vi "target_finder_3.vi"(6 "prev_count":i32, 9 "Lane_center":dbl, 10 "roi_dead":bool, 11 "Lane_center in":dbl) -> (1 "next_count":i32, 2 "Reset_ROI":dbl, 3 "Lane_center out":dbl)   [LabVIEW 2024]
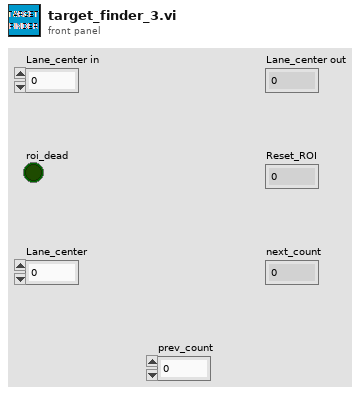
[diagram p1: front panel]
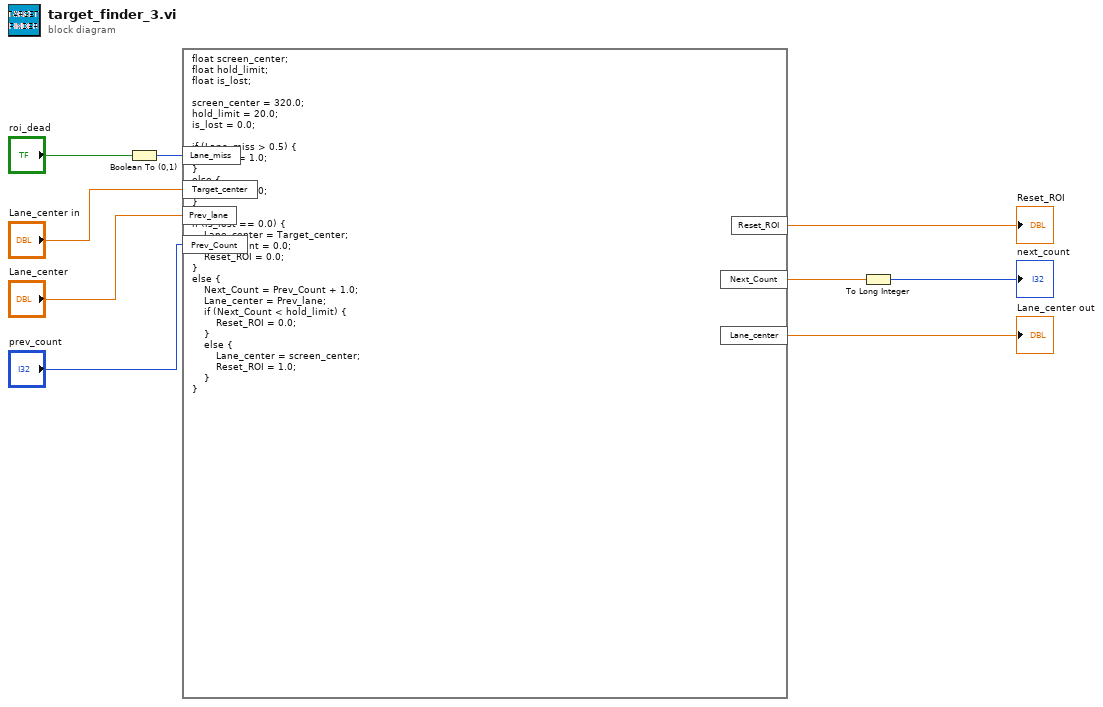
[diagram p0: block diagram]
diagram:
  n1 = Boolean To (0,1)(Boolean="roi_dead") -> (0, 1=w4:i16)
  n2 = formula code="float screen_center;\nfloat hold_limit;\nfloat is_lost;\n\nscreen_center = 320.0;\nhold_limit = 20.0;\nis_lost = 0.0;\n\nif (Lane_miss > 0.5) {\n    is_lost = 1.0;\n}\nelse {\n    is_lost = 0.0;\n}\n\nif (is_lost == 0.0) {\n    Lane_center = Target_center;\n    Next_Count = 0.0;\n    Reset_ROI = 0.0;\n}\nelse {\n    Next_Count = Prev_Count + 1.0;\n    Lane_center = Prev_lane; \n    if (Next_Count < hold_limit) {\n        Reset_ROI = 0.0;\n    }\n    else {\n        Lane_center = screen_center;\n        Reset_ROI = 1.0;\n    }\n}"("Lane_miss"=w4, "Prev_lane"="Lane_center", "Prev_Count"="prev_count", "Target_center"="Lane_center in") -> ("Reset_ROI"=→"Reset_ROI":dbl, "Next_Count"=w6:dbl, "Lane_center"=→"Lane_center out":dbl)
  n3 = To Long Integer(number=w6) -> (32bit integer=→"next_count":i32)
